vi "Lint VIs.vi"(8 "error in":errorcluster, 9 "Options":T1={"Force?"=FALSE, "Ignore List"=[], "Only List"=[], "Save(T)?"=TRUE}, 10 "Project Root Folder":path, 11 "Project Manager in":refnum<class "Project Manager.lvclass">) -> (0 "error out":errorcluster, 3 "Project Manager out":refnum<class "Project Manager.lvclass">)   [LabVIEW 2026, in "Project Manager.lvclass"]
doc: "Lint all VIs in project directory using blue."
uses:
  Project Manager.lvclass
  <vilib>/SAS/blue/blue_core/API/Options--cluster.ctl
  Project Manager.lvclass/Project Manager.ctl
  Interfaces/ILogger/ILogger Messages/Log Msg/Log Msg.lvclass/Log Msg.ctl
  <vilib>/ActorFramework/Message Enqueuer/Message Enqueuer.lvclass/Message Enqueuer.ctl
  <vilib>/ActorFramework/Message Enqueuer/Enqueue.vi
  Interfaces/ILogger/ILogger Messages/Log Msg/Log Msg.lvclass
  <vilib>/ActorFramework/Message Priority Queue/Priority Enqueue.vi
  <vilib>/SAS/blue/blue_core/API/API.lvclass
  <userlib>/_OpenG.lib/file/file.llb/openg_file.lvlib
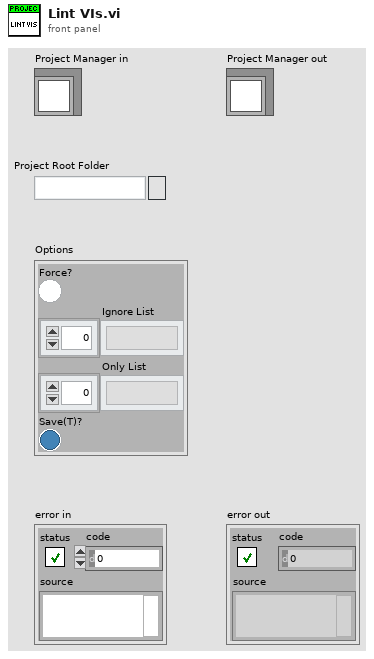
[diagram p1: front panel]
types:
  T1 = typedef "lib_blue_core.lvlib/API.lvclass/Options--cluster.ctl" = cluster{"Force?":bool, "Ignore List":string[], "Only List":string[], "Save(T)?":bool}
  T2 = typedef "lib_blue_core.lvlib/API.lvclass/Events--cluster.ctl" = cluster{"Finished Run":refnum<user-event>, "Stopped":refnum<user-event>, "Ignore Files Found":refnum<user-event>, "Processing File":refnum<user-event>, "File Saved":refnum<user-event>, "File Processed":refnum<user-event>, "Processing Error":refnum<user-event>, "Step Started":refnum<user-event>, "Step Finished":refnum<user-event>, "GUI Detected":refnum<user-event>, "Bookmarks Found":refnum<user-event>, "Steps Ignored":refnum<user-event>, "PW Protected":refnum<user-event>, "Step Skipped No BD":refnum<user-event>, "Total Files to Process":refnum<user-event>}
  T3 = typedef "Log Entry--cluster.ctl" = cluster{"Time":timestamp, "Message":string}
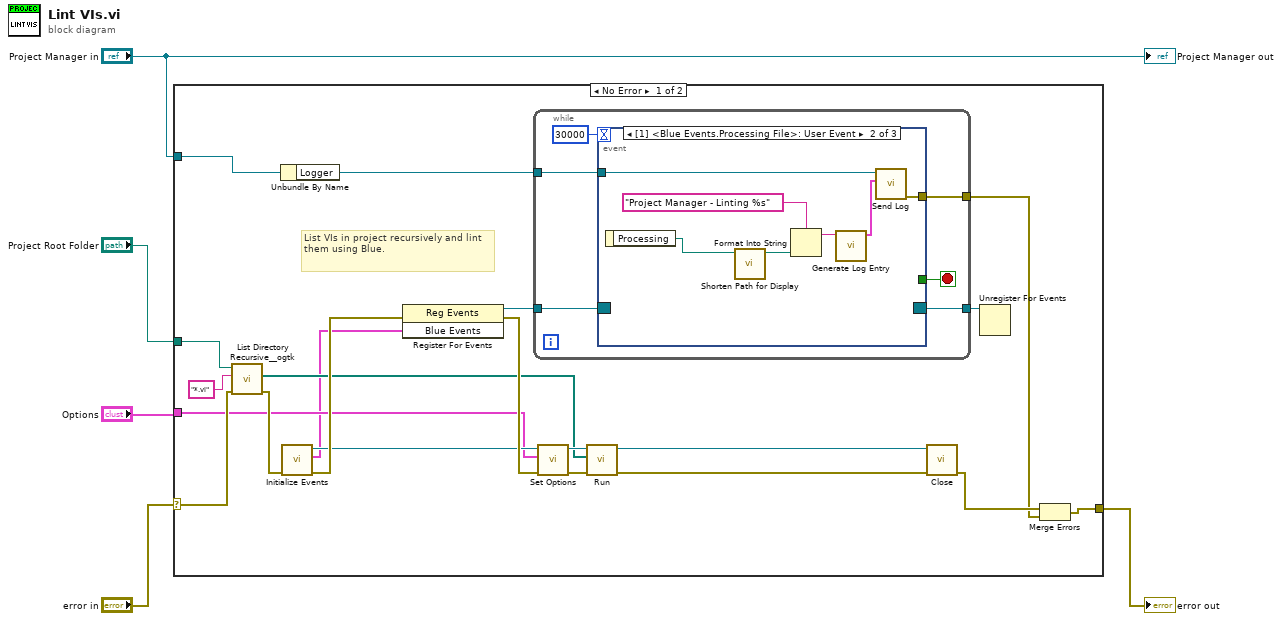
[diagram p0: block diagram]
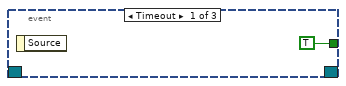
[diagram p2: hidden frame]
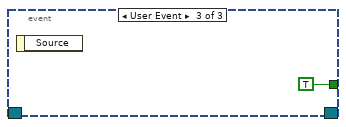
[diagram p3: hidden frame]
diagram:
  n1 = case shown="No Error" "error in" {
    selector: "error in" -> [w22 w42]
    tunnel: "Options" -> [w16 _]
    tunnel: "Project Root Folder" -> [w11 _]
    tunnel: [w19 w42] -> w5
    tunnel: "Project Manager in" -> [w8 _]
    frame No Error {
      # "List VIs in project recursively and lint them using Blue."
      n2 = call <userlib>:"List Directory Recursive__ogtk.vi"("error in (no error)"=w22, "pattern"="*.vi", "Path"=w11) -> ("error out"=w24:errorcluster, "file paths"=w13:path[])  [unwired: 5 in, 2 out]
      n3 = Unbundle By Name(w8) -> ("Logger"=w7:refnum<class "Message Enqueuer.lvclass">)
      n4 = call <vilib>:"Initialize Events.vi"("error in"=w24) -> ("error out"=w21:errorcluster, "Blue Events"=w9:T2, "API out"=w17:refnum<class "API.lvclass">)  [unwired: 8 in]
      n5 = register-events(error in=w21, w9) -> (reference out=w10:refnum<event-registration>, error out=w20:errorcluster)  [unwired: 1 in]
      n6 = while {
        tunnel: w10 -> [w31]
        tunnel: w7 -> [w30]
        tunnel: [w32] -> w18
        tunnel: [w27] -> w6
        stop <- w28 stop-if-true
        n7 = event shown="[1] <Blue Events.Processing File>: User Event" {
          selector: w31 -> [_ _ _]
          dyn-events: [_ _ _] -> w27
          timeout: 30000 -> [_ _ _]
          tunnel: w30 -> [_ w35 _]
          tunnel: [_ w40 _] -> w32
          tunnel: [TRUE _ TRUE] -> w28
          event Timeout {
            n8 = event-data() -> ()  [unwired: 1 in, 1 out]
          }
          event User Event {
            n9 = event-data() -> ("Processing"=w38:path)  [unwired: 1 in]
            n10 = call "Shorten Path for Display.vi"("Path"=w38) -> ("Shortened Path"=w37:path)  [unwired: 10 in]
            n11 = Format Into String(format string="Project Manager - Linting %s", w37) -> (resulting string=w36:string)  [unwired: 2 in, 1 out]
            n12 = call "Generate Log Entry.vi"("Message"=w36) -> ("Log Entry"=w34:T3)  [unwired: 9 in, 1 out]
            n13 = call "Send Log.vi"("Log Entry"=w34, "Message Enqueuer"=w35) -> ("error out"=w40:errorcluster)  [unwired: 8 in, 1 out]
          }
          event User Event {
            n14 = event-data() -> ()  [unwired: 1 in, 1 out]
          }
        }
      }
      n15 = call <vilib>:"Set Options.vi"("error in"=w20, "Options"=w16, "API in"=w17) -> ("error out"=w26:errorcluster, "API out"=w15:refnum<class "API.lvclass">)  [unwired: 7 in]
      n16 = call <vilib>:"Run.vi"("error in"=w26, "Absolute Paths to Process"=w13, "API in"=w15) -> ("error out"=w25:errorcluster, "API out"=w14:refnum<class "API.lvclass">)  [unwired: 7 in]
      n17 = call <vilib>:"Close.vi"("error in"=w25, "API in"=w14) -> ("error out"=w23:errorcluster)  [unwired: 9 in]
      n18 = Unregister For Events(event registration refnum=w6) -> ()  [unwired: 1 in, 1 out]
      n19 = Merge Errors(w23, w18) -> (w19:errorcluster)
    }
    frame Error {
      # "Pass error without further actions."
    }
  }
  "error out" <- w5
  "Project Manager out" <- "Project Manager in"
